vi "Update Inputs.vi"(8 "error in (no error)":errorcluster, 10 "Inputs":T1[](array[typedef]), 11 "UI Template in":refnum<class "AIO_Panel.lvclass">) -> (0 "error out":errorcluster, 3 "UI Template out":refnum<class "AIO_Panel.lvclass">)   [LabVIEW 2021, in "Simulator-Channel.lvlib" / "AIO_Panel.lvlib" / "AIO_Panel.lvclass"]
uses:
  AIO_Panel.lvclass
  tdef/info.ctl
  AIO_Panel.lvclass/AIO_Panel.ctl
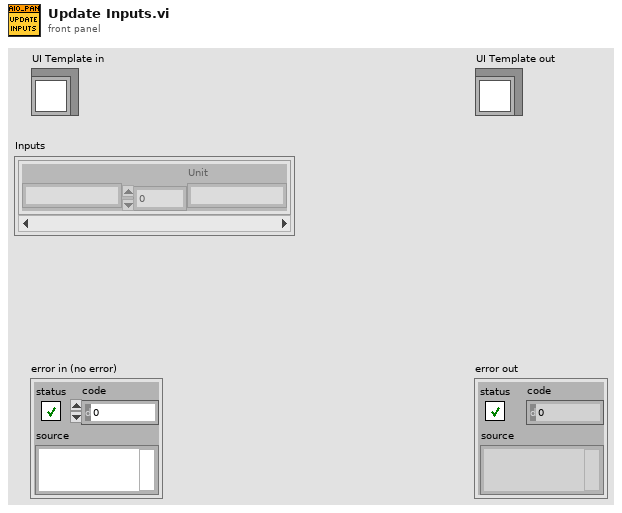
[diagram p1: front panel]
types:
  T1 = typedef "Simulator-Channel.lvlib/AIO_Panel.lvlib/AIO_Panel.lvclass/info.ctl" = cluster{"Name":string, "Numeric":dbl, "Unit":string}
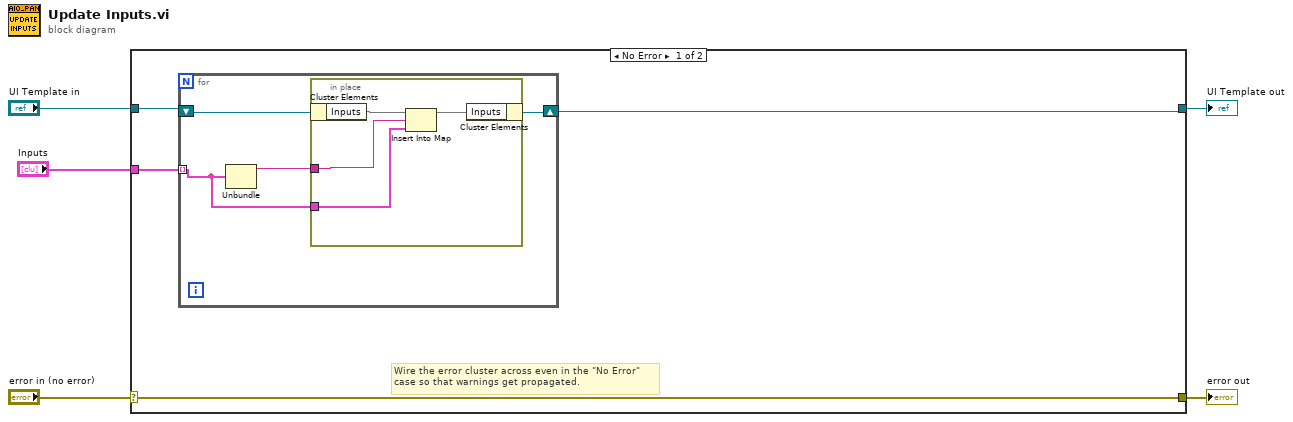
[diagram p0: block diagram]
diagram:
  n1 = case shown="No Error" "error in (no error)" {
    selector: "error in (no error)" -> [w9 w19]
    tunnel: [w9 w19] -> w4
    tunnel: [w6 w18] -> w2
    tunnel: "UI Template in" -> [w7 w18]
    tunnel: "Inputs" -> [w8 _]
    frame No Error {
      # "Wire the error cluster across even in the \"No Error\"\ncase so that warnings get propagated."
      n2 = for {
        tunnel: w8 -> [w10] mode=indexing
        shift-right: [w12] -> w6
        shift-left: w7 -> [w13]
        n3 = Unbundle(w10) -> ("Name"=w11:string)  [unwired: 2 out]
        n4 = in-place {
          in-place-border: w11 -> [w15]
          in-place-border: w10 -> [w14]
          n5 = in-place-cluster #1(w13) -> ("Inputs"=w17:map{string, T1})
          n6 = Insert Into Map(map in=w17, key=w15, value=w14) -> (map out=w16:map{string, T1})  [unwired: 2 out]
          n7 = in-place-cluster #1("Inputs"=w16) -> (w12:refnum<class "AIO_Panel.lvclass">)
        }
      }
    }
    frame Error {
    }
  }
  "error out" <- w4
  "UI Template out" <- w2
